vi "SeqEditor_StepMLSTdelete.vi"(8 "error in (no error)":errorcluster, 11 "NLTest in":refnum<class "NLTest.lvclass">) -> (0 "error out":errorcluster, 3 "NLTest out":refnum<class "NLTest.lvclass">)   [LabVIEW 2017, in "NLTest.lvclass"]
uses:
  NLTest.lvclass
  NLTest.lvclass/NLTest.ctl
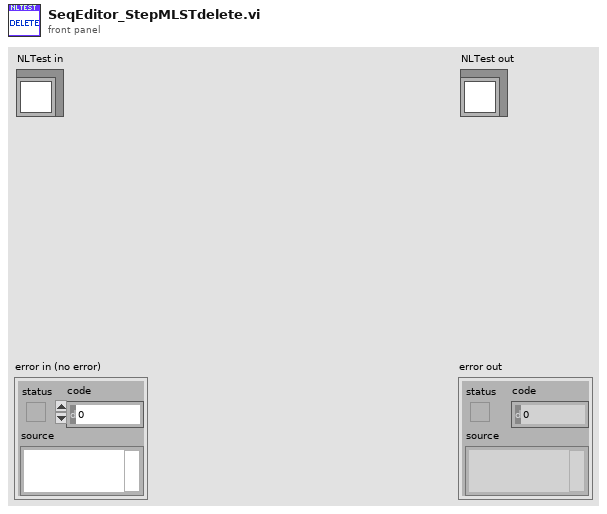
[diagram p1: front panel]
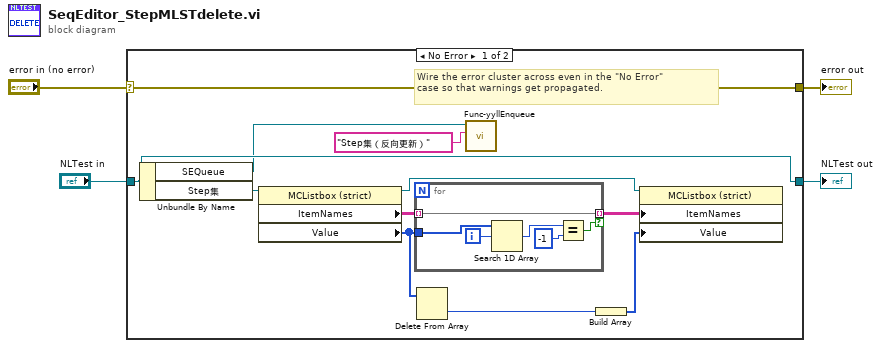
[diagram p0: block diagram]
diagram:
  n1 = case shown="No Error" "error in (no error)" {
    selector: "error in (no error)" -> [w15 w23]
    tunnel: [w15 w23] -> w3
    tunnel: [w10 w22] -> w1
    tunnel: "NLTest in" -> [w10 w22]
    frame No Error {
      # "Wire the error cluster across even in the \"No Error\"\ncase so that warnings get propagated."
      n2 = Unbundle By Name(w10) -> ("SEQueue"=w9:refnum<queue>, "Step集"=w8:refnum<vi>)
      n3 = property class="MCListbox (strict)"(reference=w8) -> (reference out=w11:refnum<vi>, "ItemNames"=w12:string[][], "Value"=w7:i32[])  [unwired: 1 in, 1 out]
      n4 = for {
        tunnel: w12 -> [w21] mode=indexing
        tunnel: w7 -> [w20]
        tunnel: [w21] -> w13 mode=indexing if=w17
        i -> [w16]
        n5 = Search 1D Array(1D array=w20, element=w16) -> (index of element=w19:i32)  [unwired: 1 in]
        n6 = Equal?(x=w19, y=-1) -> (x = y?=w17:bool)
      }
      n7 = Delete From Array(array=w7) -> (deleted portion=w6:i32)  [unwired: 2 in, 1 out]
      n8 = call "Func-yyllEnqueue.vi"("cmd"="Step集（反向更新）", "queue in"=w9) -> ()  [unwired: 7 in, 3 out]
      n9 = Build Array(w6) -> (w5:i32[])
      n10 = property class="MCListbox (strict)"(reference=w11, "ItemNames"=w13, "Value"=w5) -> ()  [unwired: 1 in, 2 out]
    }
    frame Error {
    }
  }
  "error out" <- w3
  "NLTest out" <- w1
